vi "ramptime.vi"() -> ()   [LabVIEW 2012]
panel:
  out "Setpoint vs. Time":cluster{i32[], dbl[]}(graph)
  out "Temp vs. Time":cluster{i32[], dbl[]}(graph)
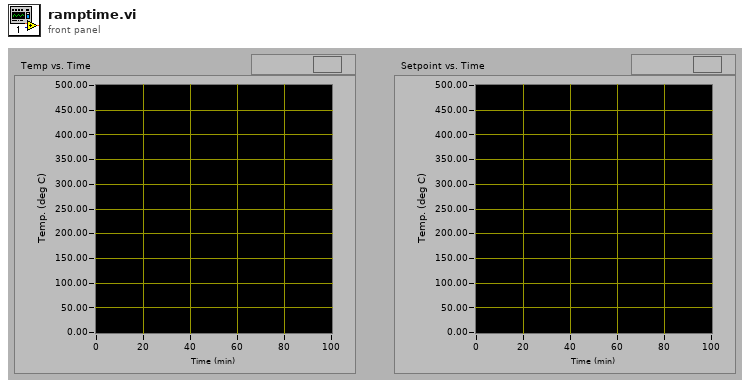
[diagram p1: front panel]
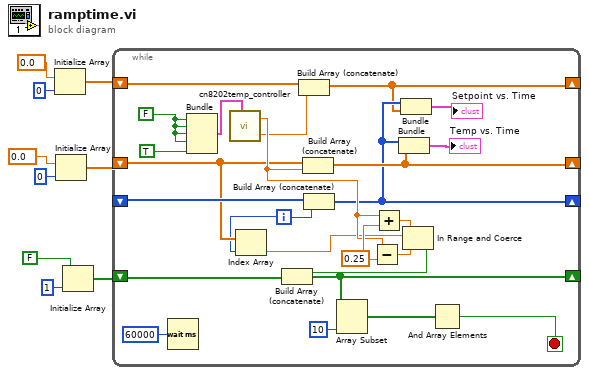
[diagram p0: block diagram]
diagram:
  n1 = Initialize Array(0.0 ("element"), 0 ("dimension size")) -> (w4:dbl[])
  n2 = Initialize Array(0.0 ("element"), 0 ("dimension size")) -> (w3:dbl[])
  n3 = Initialize Array(FALSE, 1 ("dimension size")) -> (w9:bool[])
  n4 = while {
    shift-right: [w29] -> _
    shift-left: w3 -> [w17]
    shift-right: [w11] -> _
    shift-left: _ -> [w30]
    shift-right: [w25] -> _
    shift-left: w9 -> [w20]
    shift-right: [w10] -> _
    shift-left: w4 -> [w13]
    i -> [w16]
    stop <- w22 stop-if-true
    w28 = 0.25 ("y")
    w33 = FALSE
    n5 = Wait (ms)(milliseconds to wait=u32 60000 ("millisecond multiple")) -> ()  [unwired: 1 out]
    n6 = Bundle(w33, w33, w33, w33, TRUE) -> (w34:cluster{bool, bool, bool, bool, bool})  [unwired: 1 in]
    n7 = call "cn8202temp_controller.vi"("actions"=w34) -> ("Current Recipe \nSetpoint (deg C)"=w14:dbl, "Thermometer"=w18:dbl)  [unwired: 5 in]
    n8 = Index Array(array=w17, index=w16) -> (element=w15:dbl)
    n9 = Build Array (concatenate)(w13, w14) -> (w10:dbl[])
    n10 = Build Array (concatenate)(w17, w18) -> (w29:dbl[])
    n11 = Build Array (concatenate)(w30, w16) -> (w11:i32[])
    n12 = Subtract(x=w18, y=w28) -> (x-y=w26:dbl)
    n13 = Add(x=w18, y=w28) -> (x+y=w27:dbl)
    n14 = Bundle(w11, w29) -> (→"Temp vs. Time":cluster{i32[], dbl[]})  [unwired: 1 in]
    n15 = Bundle(w11, w10) -> (→"Setpoint vs. Time":cluster{i32[], dbl[]})  [unwired: 1 in]
    n16 = In Range and Coerce(upper limit=w27, x=w15, lower limit=w26) -> (In Range?=w21:bool)  [unwired: 1 out]
    n17 = Build Array (concatenate)(w21, w20) -> (w25:bool[])
    n18 = Array Subset(array=w25, length=10) -> (w23:bool[])  [unwired: 1 in]
    n19 = And Array Elements(Boolean array=w23) -> (logical AND=w22:bool)
  }
